vi "set Trigger Source.vi"(8 "error in (no error)":errorcluster, 10 "Trigger Source":T1(ring), 11 "Keysight 9020A in":refnum<class "Keysight 9020A.lvclass">) -> (0 "error out":errorcluster, 3 "Keysight 9020A out":refnum<class "Keysight 9020A.lvclass">)   [LabVIEW 2023, in "Spectrum Analyzer.lvlib" / "Keysight 9020A.lvclass"]
uses:
  Keysight 9020A.lvclass
  Keysight 9020A.lvclass/Keysight 9020A.ctl
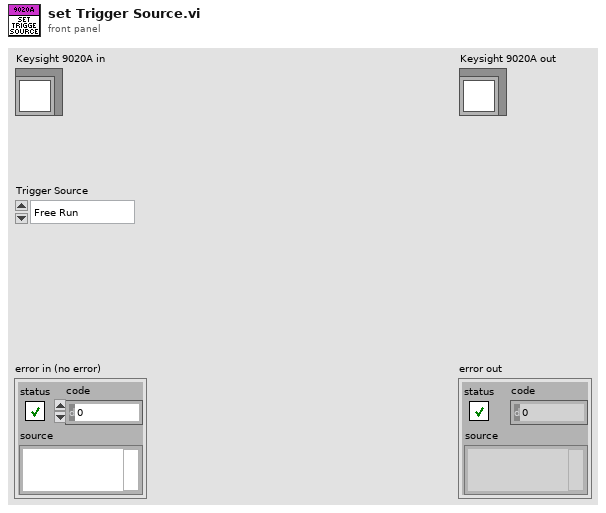
[diagram p1: front panel]
types:
  T1 = enum16{"Free Run", "Video (IF Envelop)", "RF Burst"}
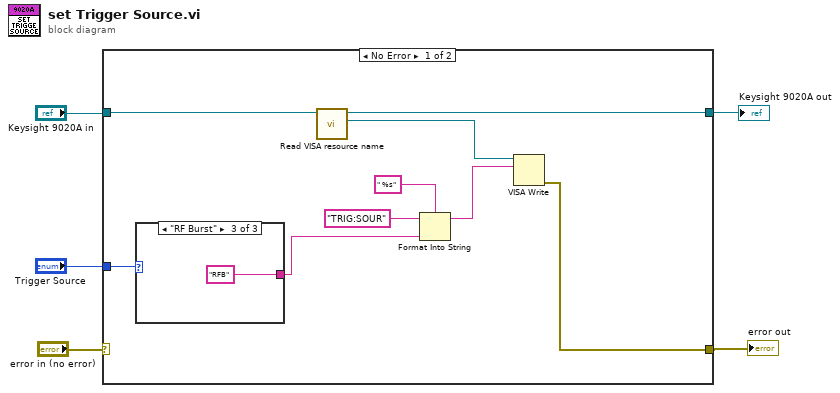
[diagram p0: block diagram]
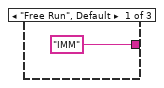
[diagram p2: hidden frame]
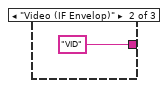
[diagram p3: hidden frame]
diagram:
  n1 = case shown="No Error" "error in (no error)" {
    selector: "error in (no error)" -> [_ w18]
    tunnel: "Keysight 9020A in" -> [w9 w19]
    tunnel: [w14 w19] -> w4
    tunnel: [w10 w18] -> w2
    tunnel: "Trigger Source" -> [w7 _]
    frame No Error {
      n2 = case shown="\"RF Burst\"" w7 {
        tunnel: ["IMM" "VID" "RFB"] -> w6
        frame "Free Run", Default {
        }
        frame "Video (IF Envelop)" {
        }
        frame "RF Burst" {
        }
      }
      n3 = call "Read VISA resource name.vi"("Keysight 9020A in"=w9) -> ("VISA resource name"=w12:refnum<visa-resource-name>, "Keysight 9020A out"=w14:refnum<class "Keysight 9020A.lvclass">)  [unwired: 8 in, 1 out]
      n4 = Format Into String(format string=" %s", initial string="TRIG:SOUR", w6) -> (resulting string=w11:string)  [unwired: 1 in, 1 out]
      n5 = VISA Write(VISA resource name=w12, write buffer=w11) -> (error out=w10:errorcluster)  [unwired: 1 in, 2 out]
    }
    frame Error {
    }
  }
  "error out" <- w2
  "Keysight 9020A out" <- w4
